vi "Main.vi"() -> ()   [LabVIEW 2026]
doc: "Use this template to build a producer/consumer design pattern. Use this template when you need to execute a process, such as data analysis, when a data source, such as a triggered acquisition, produces data at an uneven rate and you need to execute the process when the data becomes available."
uses:
  Measurement_Data.ctl
panel:
  out "Last_SMS_Message":variant
  out "SMS_Message_Previev":string
  out "Send_Notification":bool
  out "Water_Alarm":bool
  out "Humidity_Alarm":bool
  out "Temperature_alarm":bool
  in  "Humidity_Limit":dbl
  in  "Temperature_Limit":dbl
  in  "Parameter":u16(ring) items=["Temperature", "Humidity", "Pressure"]
  out "Waveform Chart":dbl(graph)
  out "Timestamp":timestamp
  out "Water_detected":bool
  out "Pressure":dbl
  out "Humidity":dbl
  out "Temperature":dbl
  in  "stop":bool
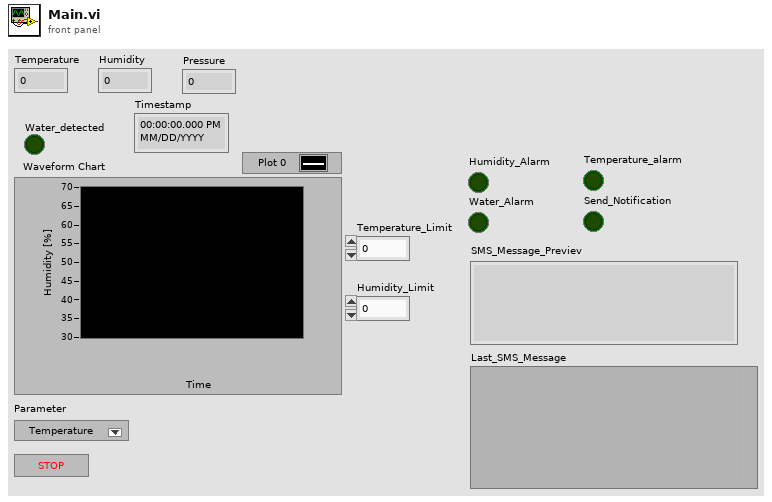
[diagram p1: front panel]
types:
  T1 = typedef "Measurement_Data.ctl" = cluster{"Temperature":dbl, "Humidity":dbl, "Pressure":dbl, "Water_detected":bool, "Timestamp":timestamp}
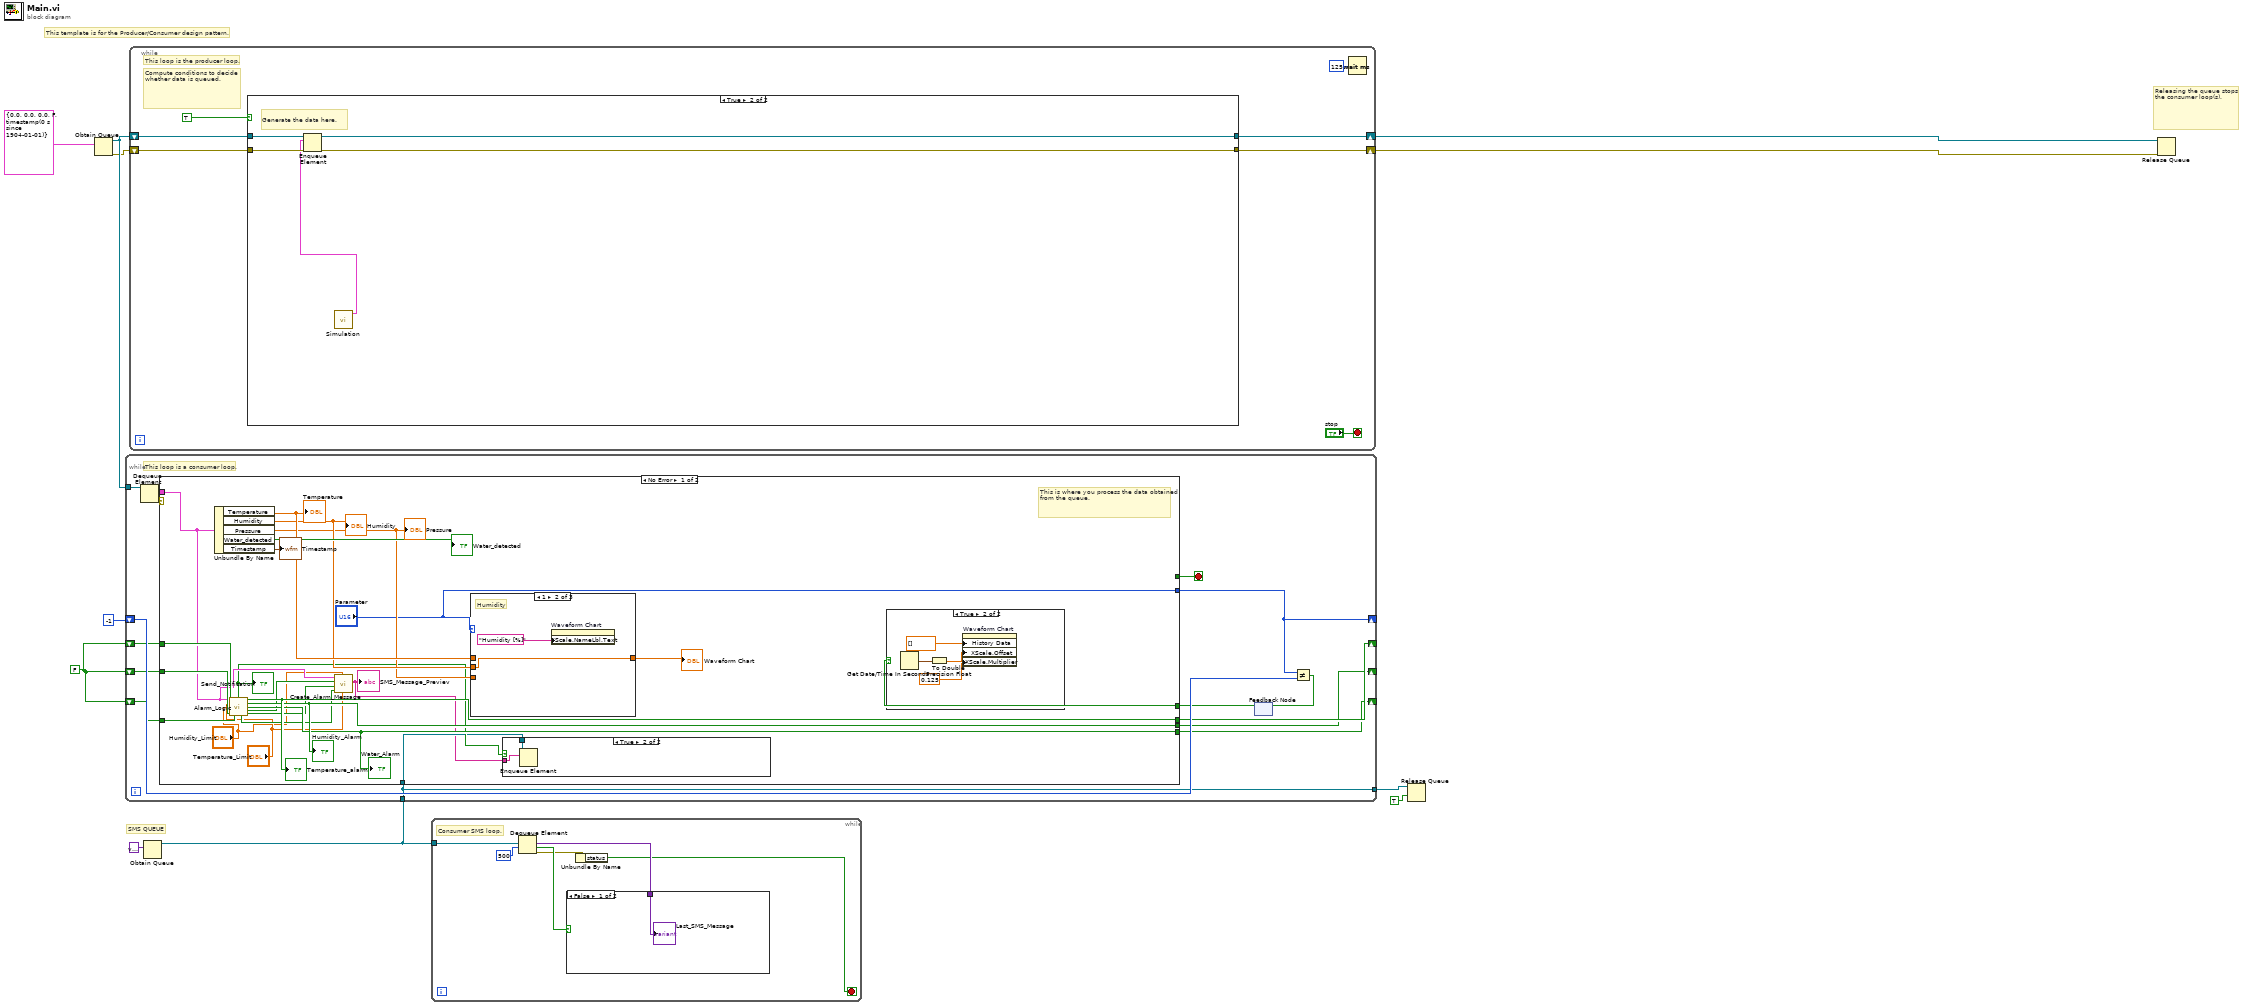
[diagram p0: block diagram]
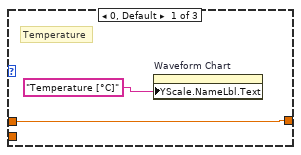
[diagram p5: hidden frame]
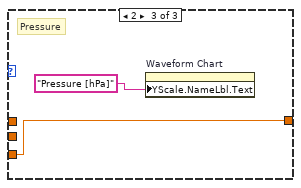
[diagram p6: hidden frame]
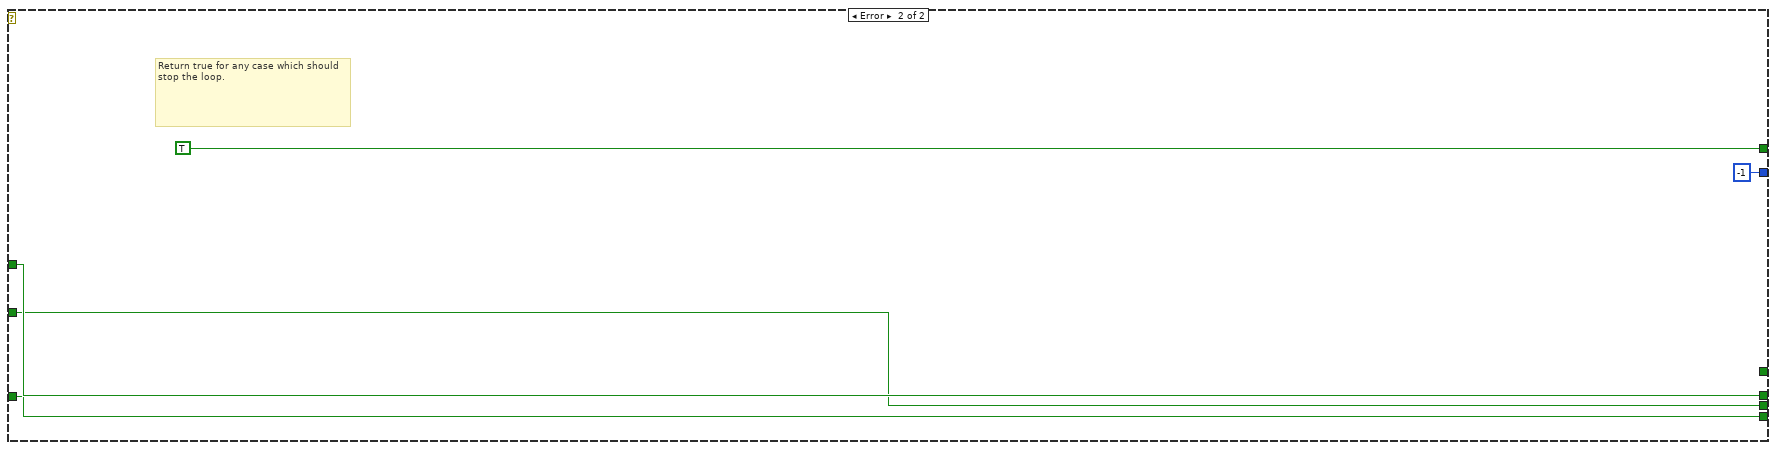
[diagram p7: hidden frame]
diagram:
  w5 = FALSE
  # "SMS QUEUE"
  # "Releasing the queue stops the consumer loop(s)."
  # "This template is for the Producer/Consumer design pattern."
  n1 = Obtain Queue(element data type=T1 {"Temperature"=0.0, "Humidity"=0.0, "Pressure"=0.0, "Water_detected"=FALSE, "Timestamp"=timestamp(0 s since 1904-01-01)} ("Measurement_Data")) -> (queue out=w11:refnum<queue>, error out=w10:errorcluster)  [unwired: 4 in, 1 out]
  n2 = while {
    shift-right: [w14] -> w8
    shift-left: w10 -> [w15]
    shift-right: [w16] -> w9
    shift-left: w11 -> [w17]
    stop <- "stop" stop-if-true
    # "Compute conditions to decide whether data is queued."
    # "This loop is the producer loop."
    n3 = case shown="True" TRUE ("Case Constant\n(See Context Help)") {
      tunnel: w17 -> [w20 w25]
      tunnel: [w20 w24] -> w16
      tunnel: w15 -> [w19 w23]
      tunnel: [w19 w22] -> w14
      frame False {
      }
      frame True {
        # "Generate the data here."
        n4 = call "Simulation.vi"() -> ("Measurement_Data out"=w21:T1)  [unwired: 11 in]
        n5 = Enqueue Element(queue=w25, element=w21, error in (no error)=w23) -> (queue out=w24:refnum<queue>, error out=w22:errorcluster)  [unwired: 1 in, 1 out]
      }
    }
    n6 = Wait (ms)(milliseconds to wait=u32 125) -> ()  [unwired: 1 out]
  }
  n7 = Obtain Queue(element data type=variant) -> (queue out=w3:refnum<queue>)  [unwired: 4 in, 2 out]
  n8 = while {
    tunnel: w11 -> [w40]
    shift-right: [w33] -> _
    shift-left: -1 -> [w36]
    shift-right: [w29] -> _
    shift-left: w5 -> [w32]
    shift-right: [w28] -> _
    shift-left: w5 -> [w31]
    shift-right: [w27] -> _
    shift-left: w5 -> [w30]
    tunnel: w3 -> [w26]
    tunnel: [w26] -> w2
    stop <- w37 stop-if-true
    # "This loop is a consumer loop."
    n9 = Dequeue Element(queue=w40) -> (element=w38:T1, error out=w39:errorcluster)  [unwired: 2 in, 2 out]
    n10 = feedback #1() -> (w34:bool)  [unwired: 1 in]
    n11 = case shown="No Error" w39 {
      tunnel: w38 -> [w46 _]
      tunnel: [_ TRUE] -> w37
      tunnel: ["Parameter" i8 -1 ("Parameter")] -> w33
      tunnel: w34 -> [w56 _]
      tunnel: w32 -> [w55 w78]
      tunnel: w31 -> [w54 w77]
      tunnel: w30 -> [w53 w76]
      tunnel: [w52 w78] -> w29
      tunnel: [w51 w77] -> w28
      tunnel: [w50 w76] -> w27
      tunnel: w26 -> [w42 _]
      frame No Error {
        # "This is where you process the data obtained from the queue."
        n12 = Unbundle By Name(w46) -> ("Temperature"=w61:dbl, "Humidity"=w59:dbl, "Pressure"=w58:dbl, "Water_detected"=→"Water_detected":bool, "Timestamp"=→"Timestamp":timestamp)
        "Temperature" <- w61
        "Humidity" <- w59
        "Pressure" <- w58
        n13 = call "Alarm_Logic.vi"("Measurement_Data"=w46, "Temperature_Limit"="Temperature_Limit", "Humidity_Limit"="Humidity_Limit", "Previous_Temperature_Alarm"=w55, "Previous_Humidity_Alarm"=w54, "Previous_Water_Alarm"=w53) -> ("Send_Notification"=w43:bool, "Temperature_Alarm"=w52:bool, "Humidity_Alarm"=w51:bool, "Water_Alarm"=w50:bool, "New_Temperature_Alarm"=w49:bool, "New_Water_Alarm"=w47:bool, "New_Humidity_Alarm"=w48:bool)  [unwired: 3 in]
        "Temperature_alarm" <- w52
        "Humidity_Alarm" <- w51
        "Water_Alarm" <- w50
        "Send_Notification" <- w43
        n14 = call "Create_Alarm_Message.vi"("Temperature_Limit"="Temperature_Limit", "Humidity_Limit"="Humidity_Limit", "New_Water_Alarm"=w47, "New_Humidity_Alarm"=w48, "New_Temperteture_Alarm"=w49, "Measurement_Data"=w46) -> ("SMS_Message"=w41:string)  [unwired: 5 in]
        "SMS_Message_Previev" <- w41
        n15 = case shown="1" "Parameter" {
          tunnel: w61 -> [w71 _ _]
          tunnel: [w71 w73 w75] -> w60
          tunnel: w59 -> [_ w73 _]
          tunnel: w58 -> [_ _ w75]
          frame 0, Default {
            # "Temperature"
            n16 = property on="Waveform Chart" class="WFChart (strict)"("YScale.NameLbl.Text"="Temperature [°C]") -> ()  [unwired: 2 in, 2 out]
          }
          frame 1 {
            # "Humidity"
            n17 = property on="Waveform Chart" class="WFChart (strict)"("YScale.NameLbl.Text"="Humidity [%]") -> ()  [unwired: 2 in, 2 out]
          }
          frame 2 {
            # "Pressure"
            n18 = property on="Waveform Chart" class="WFChart (strict)"("YScale.NameLbl.Text"="Pressure [hPa]") -> ()  [unwired: 2 in, 2 out]
          }
        }
        "Waveform Chart" <- w60
        n19 = case shown="True" w43 {
          tunnel: w42 -> [_ w65]
          tunnel: w41 -> [_ w64]
          frame False {
          }
          frame True {
            n20 = Enqueue Element(queue=w65, element=w64) -> ()  [unwired: 2 in, 3 out]
          }
        }
        n21 = case shown="True" w56 {
          frame False {
          }
          frame True {
            n22 = Get Date/Time In Seconds() -> (seconds since 1Jan1904=w68:timestamp)
            n23 = To Double Precision Float(number=w68) -> (double precision float=w67:dbl)
            n24 = property on="Waveform Chart" class="WFChart (strict)"("History Data"=dbl[] [], "XScale.Offset"=w67, "XScale.Multiplier"=0.125 ("X Scale.Offset and Multiplier:Multiplier")) -> ()  [unwired: 2 in, 2 out]
          }
        }
      }
      frame Error {
        # "Return true for any case which should stop the loop."
      }
    }
    n25 = Not Equal?(x=w33, y=w36) -> (x != y?=w35:bool)
    n26 = feedback-in #1(w35) -> ()
  }
  n27 = while {
    tunnel: w3 -> [w86]
    stop <- w81 stop-if-true
    # "Consumer SMS loop."
    n28 = Dequeue Element(queue=w86, timeout in ms (-1)=500) -> (element=w83:variant, timed out?=w84:bool, error out=w82:errorcluster)  [unwired: 1 in, 1 out]
    n29 = case shown="False" w84 {
      tunnel: w83 -> [w87 _]
      frame False {
        "Last_SMS_Message" <- w87
      }
      frame True {
      }
    }
    n30 = Unbundle By Name(w82) -> ("status"=w81:bool)
  }
  n31 = Release Queue(queue=w2, force destroy? (F)=TRUE) -> ()  [unwired: 1 in, 3 out]
  n32 = Release Queue(queue=w9, error in (no error)=w8) -> ()  [unwired: 1 in, 3 out]
